vi "USBTC08StreamingGetTemp.vi"(6 "Units":enum16{"C°", "F°", "K°", "R°"}(ring), 7 "Channel Enable Array":u8[](array[numeric]), 8 "error in (no error)":errorcluster, 10 "Buffer size":i32, 11 "Handle in":i16) -> (0 "error out":errorcluster, 1 "Overflow":i16[](array[numeric]), 2 "Array out":sgl[][](array[numeric]), 3 "Handle out":i16)   [LabVIEW 2009]
uses:
  usbtc08.dll
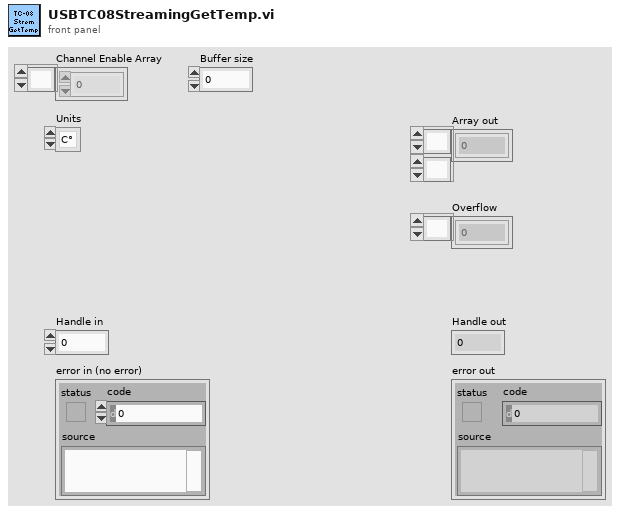
[diagram p1: front panel]
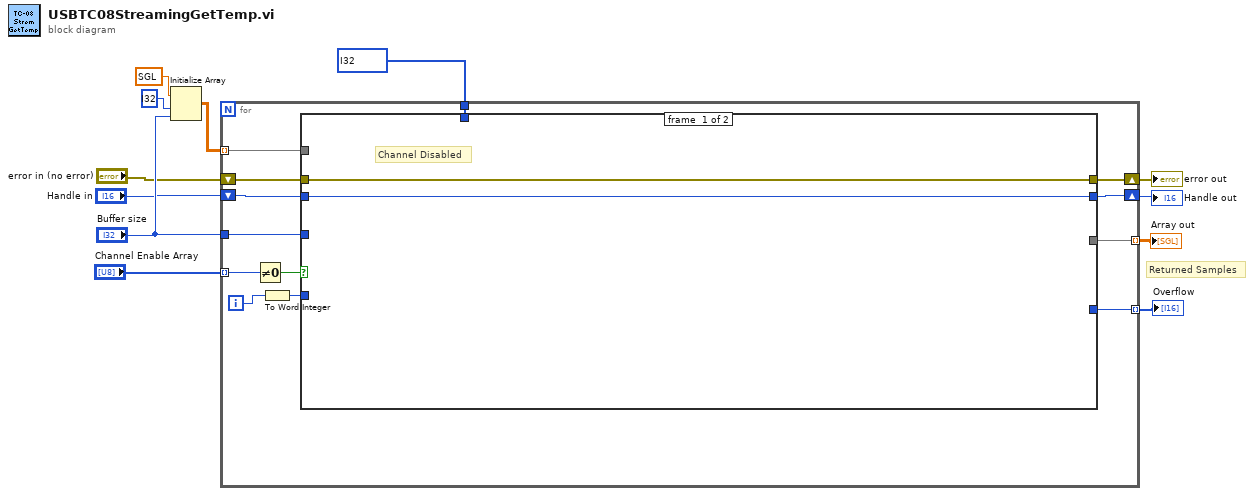
[diagram p0: block diagram]
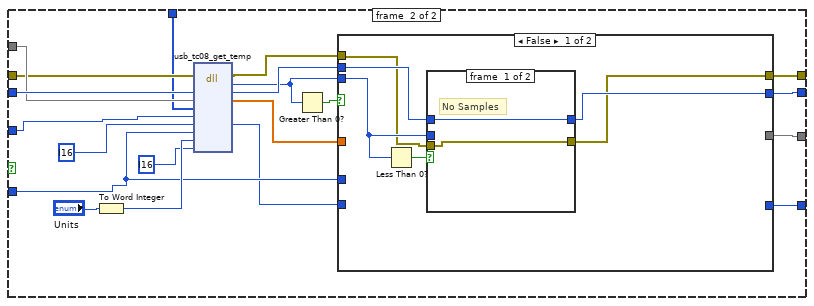
[diagram p2: hidden frame]
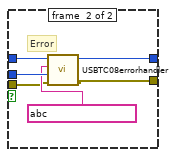
[diagram p3: hidden frame]
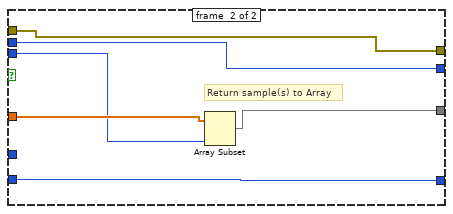
[diagram p4: hidden frame]
diagram:
  # "Returned Samples"
  n1 = Initialize Array(sgl ?, i32 ? ("dimension size"), "Buffer size") -> (w7:sgl[][])
  n2 = for {
    shift-right: [w24] -> w4
    shift-left: "Handle in" -> [w25]
    tunnel: "Channel Enable Array" -> [w22] mode=indexing
    tunnel: "Buffer size" -> [w19]
    tunnel: w7 -> [w18] mode=indexing
    tunnel: [w17] -> w9 mode=indexing
    shift-right: [w15] -> w11
    shift-left: "error in (no error)" -> [w16]
    tunnel: [w14] -> w2 mode=indexing
    tunnel: i32[] ? ("times_ms_buffer") -> [w13]
    i -> [w21]
    n3 = Not Equal To 0?(x=w22) -> (x != 0?=w23:bool)
    n4 = To Word Integer(number=w21) -> (16bit integer=w20:i16)
    n5 = case shown="True" w23 {
      tunnel: w25 -> [w27 w47]
      tunnel: [w27 w42] -> w24
      tunnel: w20 -> [_ w37]
      tunnel: w19 -> [_ w36]
      tunnel: w18 -> [_ w35]
      tunnel: [_ w34] -> w17
      tunnel: w16 -> [w26 w33]
      tunnel: [w26 w32] -> w15
      tunnel: [_ w29] -> w14
      tunnel: w13 -> [_ w28]
      frame #0 {
        # "Channel Disabled"
      }
      frame #1 {
        n6 = To Word Integer(number="Units") -> (16bit integer=w45:i16)
        n7 = dll-call lib="usbtc08.dll" fn="usb_tc08_get_temp"(error in=w33, "handle"=w47, "temp_buffer"=w35, "times_ms_buffer"=w28, "buffer_length"=w36, "overflow"=i16 ?, "channel"=w37, "units"=w45, "fill_missing"=i16 ?) -> (error out=w31:errorcluster, "return type"=w39:i32, "handle"=w40:i16, "temp_buffer"=w38:sgl[], "overflow"=w30:i16)  [unwired: 7 in, 1 out]
        n8 = Greater Than 0?(x=w39) -> (x > 0?=w41:bool)
        n9 = case shown="False" w41 {
          tunnel: w39 -> [w50 w64]
          tunnel: w40 -> [w53 w67]
          tunnel: [w52 w67] -> w42
          tunnel: w38 -> [_ w66]
          tunnel: w37 -> [_ _]
          tunnel: [_ w65] -> w34
          tunnel: [w48 w63] -> w32
          tunnel: w31 -> [w49 w63]
          tunnel: w30 -> [_ w62]
          tunnel: [_ w62] -> w29
          frame #0 {
            n10 = Less Than 0?(x=w50) -> (x < 0?=w51:bool)
            n11 = case shown="True" w51 {
              tunnel: w50 -> [_ w61]
              tunnel: w53 -> [w55 w60]
              tunnel: [w55 w59] -> w52
              tunnel: w49 -> [w54 w57]
              tunnel: [w54 w56] -> w48
              frame #0 {
                # "No Samples"
              }
              frame #1 {
                # "Error"
                n12 = call "USBTC08errorhandler.vi"("error in (no error)"=w57, "Return"=w61, "API function"=string ?, "Handle in"=w60) -> ("error out"=w56:errorcluster, "Handle out"=w59:i16)  [unwired: 6 in]
              }
            }
          }
          frame #1 {
            # "Return sample(s) to Array"
            n13 = Array Subset(array=w66, length=w64) -> (w65:sgl[])  [unwired: 1 in]
          }
        }
      }
    }
  }
  "error out" <- w11
  "Array out" <- w9
  "Handle out" <- w4
  "Overflow" <- w2
